vi "libssh2_channel_signal_ex.vi"(8 "error in (no error)":errorcluster, 10 "signal name":string, 11 "channel":T1) -> (0 "error out":errorcluster)   [LabVIEW 2017, in "libssh2.lvlib"]
doc: "Send a signal (without \"SIG\" prefix) to a process previously opened on the channel.\n\nSignals depend on the OS of the SSH server and may be ignored.\n\nFor example:\n\"TERM\" - terminate the process.\n\"IGN\" - ignore the signal (no-op).\n\"CORE\" - terminate the process and dump core.\n\"STOP\" - stop the process.\n\"CONT\" - continue the process if it is currently stopped."
uses:
  libssh2.lvlib
  Channel Refnum.ctl
  Acquire Session.vi
  Release Session.vi
  Not A Channel.vi
  <vilib>/Utility/error.llb/Error Cluster From Error Code.vi
  Global Settings.vi
  Read Channel Refnum.vi
  Read Session Refnum.vi
  <vilib>/Utility/semaphor.llb/Acquire Semaphore.vi
  <vilib>/Utility/semaphor.llb/Release Semaphore.vi
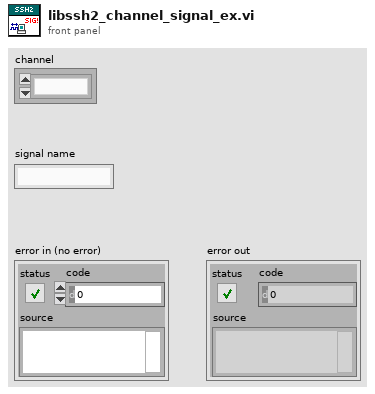
[diagram p1: front panel]
types:
  T1 = typedef "libssh2.lvlib/Channel Refnum.ctl" = refnum<k1>
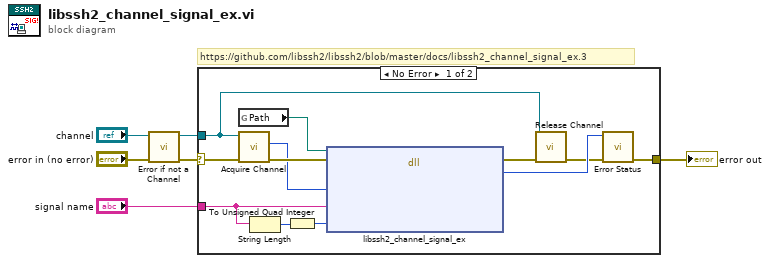
[diagram p0: block diagram]
diagram:
  # "https://github.com/libssh2/libssh2/blob/master/docs/libssh2_channel_signal_ex.3"
  n1 = call "Error if not a Channel.vi"("error in (no error)"="error in (no error)", "channel"="channel") -> ("error out"=w4:errorcluster, "channel out"=w2:T1)  [unwired: 8 in]
  n2 = case shown="No Error" w4 {
    selector: w4 -> [w18 w19]
    tunnel: [w17 w19] -> w6
    tunnel: w2 -> [w7 _]
    tunnel: "signal name" -> [w11 _]
    frame No Error {
      n3 = global read "Global Settings.vi" "Path"() -> (w13:path)
      n4 = call "Acquire Channel.vi"("error in (no error)"=w18, "channel"=w7) -> ("error out"=w15:errorcluster, "LIBSSH2_CHANNEL*"=w14:u64)  [unwired: 8 in]
      n5 = String Length(string=w11) -> (length=w10:i32)
      n6 = To Unsigned Quad Integer(1:w10) -> (0:w9:u64)
      n7 = dll-call lib="?" fn="libssh2_channel_signal_ex"(path in=w13, error in=w15, "channel"=w14, "signame"=w11, "signame_len"=w9) -> (error out=w16:errorcluster, "return value"=w12:i32)  [unwired: 4 in, 1 out]
      n8 = call "Release Channel.vi"("error in (no error)"=w16, "channel"=w7) -> ("error out"=w8:errorcluster)  [unwired: 9 in]
      n9 = call "Error Status.vi"("error in (no error)"=w8, "return value"=w12) -> ("error out"=w17:errorcluster)  [unwired: 8 in, 1 out]
    }
    frame Error {
    }
  }
  "error out" <- w6
